vi "Execute.vi"(8 "error in (no error)":errorcluster, 11 "Node in":refnum<class "bt_Repeat Until Count.lvclass">) -> (0 "error out":errorcluster, 1 "Status":T1, 3 "Node out":refnum<class "bt_Repeat Until Count.lvclass">)   [LabVIEW 2021, in "BT.lvlib" / "bt_Repeat Until Count.lvclass"]
uses:
  bt_Repeat Until Count.lvclass
  abs_Node/Status.ctl
  bt_Repeat Until Count.lvclass/bt_Repeat Until Count.ctl
  Repeater/bt_Repeater.lvclass
  abs_Node/bt_Node.lvclass
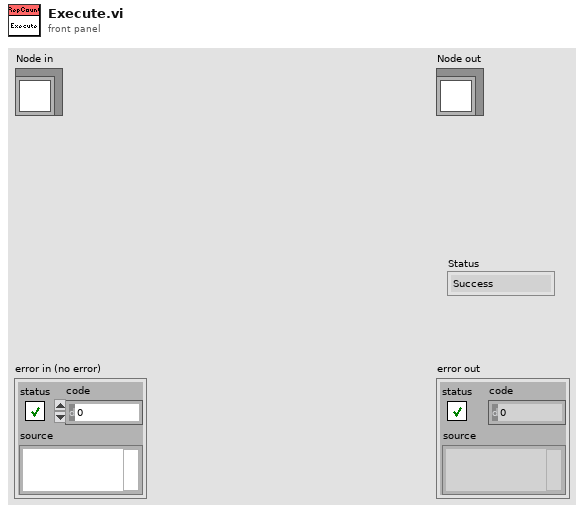
[diagram p1: front panel]
types:
  T1 = typedef "BT.lvlib/bt_Node.lvclass/Status.ctl" = enum16{"Success", "Failure", "Running"}
  T2 = typedef "BT.lvlib/bt_Repeat Until Count.lvclass/On Count Status - Type.ctl" = enum16{"Success", "Failure"}
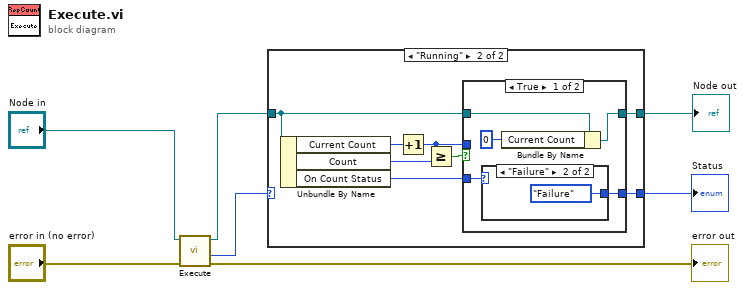
[diagram p0: block diagram]
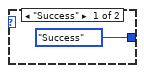
[diagram p3: hidden frame]
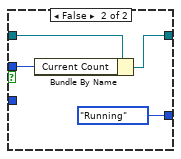
[diagram p4: hidden frame]
diagram:
  n1 = call-parent "Execute.vi"("error in (no error)"="error in (no error)", "Node in"="Node in") -> ("error out"=→"error out":errorcluster, "Status"=w1:T1, "Node out"=w2:refnum<class "bt_Repeat Until Count.lvclass">)  [unwired: 7 in]
  n2 = case shown="\"Running\"" w1 {
    selector: w1 -> [w9 _]
    tunnel: w2 -> [w8 w14]
    tunnel: [w9 w10] -> w4
    tunnel: [w8 w13] -> w3
    frame Default {
    }
    frame "Running" {
      n3 = Unbundle By Name(w14) -> ("Current Count"=w17:i32, "Count"=w16:i32, "On Count Status"=w11:T2)
      n4 = Increment(x=w17) -> (x+1=w12:i32)
      n5 = Greater Or Equal?(x=w12, y=w16) -> (x >= y?=w15:bool)
      n6 = case shown="True" w15 {
        tunnel: w14 -> [w22 w28]
        tunnel: [w21 w27] -> w13
        tunnel: w12 -> [_ w26]
        tunnel: w11 -> [w19 _]
        tunnel: [w18 Status."Running" ("Status")] -> w10
        frame True {
          n7 = case shown="\"Failure\"" w19 {
            tunnel: [Status."Success" ("Status") Status."Failure" ("Status")] -> w18
            frame "Success" {
            }
            frame "Failure" {
            }
          }
          n8 = Bundle By Name(cluster=w22, "Current Count"=0) -> (w21:refnum<class "bt_Repeat Until Count.lvclass">)
        }
        frame False {
          n9 = Bundle By Name(cluster=w28, "Current Count"=w26) -> (w27:refnum<class "bt_Repeat Until Count.lvclass">)
        }
      }
    }
  }
  "Node out" <- w3
  "Status" <- w4
